vi "libssh2_session_block_directions.vi"(8 "error in (no error)":errorcluster, 11 "session":T2) -> (0 "error out":errorcluster, 2 "block direction":T1 items=["Inbound"=1, "Outbound"=2])   [LabVIEW 2017, in "libssh2.lvlib"]
doc: "Set the blocking mode for a session.\n\nWhen any of the libssh2 functions return <B>LIBSSH2_ERROR_EAGAIN</B>, a caller should wait for the socket to have data available for reading or writing before calling the function again."
uses:
  libssh2.lvlib
  Session Refnum.ctl
  libssh2_session_block_direction.ctl
  Global Settings.vi
  Read Session Refnum.vi
  <vilib>/Utility/semaphor.llb/Acquire Semaphore.vi
  <vilib>/Utility/semaphor.llb/Release Semaphore.vi
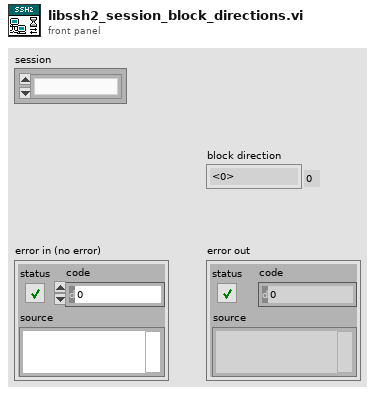
[diagram p1: front panel]
types:
  T1 = typedef "libssh2.lvlib/libssh2_session_block_direction.ctl" = i32
  T2 = typedef "libssh2.lvlib/Session Refnum.ctl" = refnum<k1>
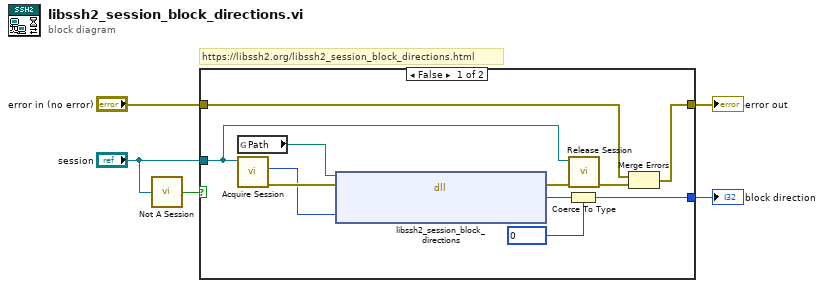
[diagram p0: block diagram]
diagram:
  # "https://libssh2.org/libssh2_session_block_directions.html"
  n1 = call "Not A Session.vi"("session"="session") -> ("Not a Session?"=w1:bool)
  n2 = case shown="False" w1 {
    tunnel: [w14 w17] -> w5
    tunnel: [w10 _] -> w4
    tunnel: "error in (no error)" -> [w8 w17]
    tunnel: "session" -> [w6 _]
    frame False {
      w9 = T1 0 items=["Inbound"=1, "Outbound"=2] ("Ring")
      n3 = global read "Global Settings.vi" "Path"() -> (w12:path)
      n4 = call "Acquire Session.vi"("session"=w6) -> ("error out"=w16:errorcluster, "LIBSSH2_SESSION*"=w15:u64)  [unwired: 8 in, 1 out]
      n5 = dll-call lib="?" fn="libssh2_session_block_directions"(path in=w12, error in=w16, "session"=w15) -> (error out=w13:errorcluster, "return value"=w11:i32)  [unwired: 2 in, 1 out]
      n6 = Coerce To Type(0:w11, 1:w9) -> (2:w10:T1)
      n7 = call "Release Session.vi"("error in (no error)"=w13, "session"=w6) -> ("error out"=w7:errorcluster)  [unwired: 9 in]
      n8 = Merge Errors(w8, w7) -> (w14:errorcluster)
    }
    frame True {
    }
  }
  "error out" <- w5
  "block direction" <- w4
